vi "Set Output.vi"(8 "error in (no error)":errorcluster, 9 "Set Output":dbl, 10 "AIO_CFG":refnum<class "AIO-Configuration.lvclass">, 11 "UI Template in":refnum<class "AIO_Panel.lvclass">) -> (0 "error out":errorcluster, 3 "UI Template out":refnum<class "AIO_Panel.lvclass">)   [LabVIEW 2021, in "Simulator-Channel.lvlib" / "AIO_Panel.lvlib" / "AIO_Panel.lvclass"]
uses:
  AIO_Panel.lvclass
  Dependencies/AIO-Channel.lvlibp/Channels/AIO-Channel/AIO-Configuration_class/AIO-Configuration.lvclass
  C:/Users/averna/Documents/LV Gym DEMO/Factory Pattern/Device Channels/Dependencies/AIO-Channel.lvlibp/Generic Channel/Channel/Configuration_class/Configuration.lvclass
  tdef/info.ctl
  AIO_Panel.lvclass/AIO_Panel.ctl
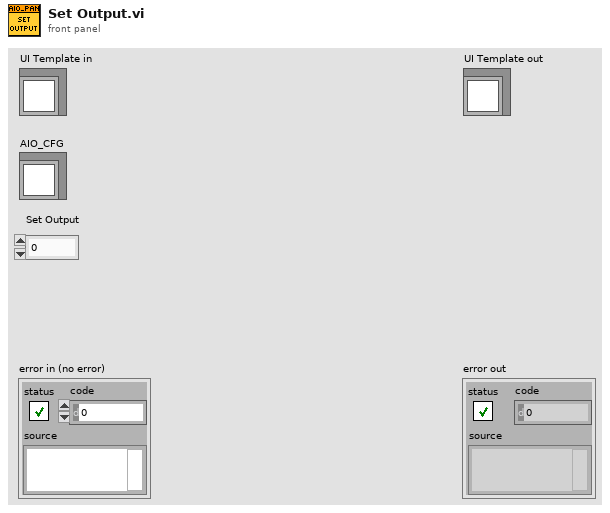
[diagram p1: front panel]
types:
  T1 = typedef "Simulator-Channel.lvlib/AIO_Panel.lvlib/AIO_Panel.lvclass/info.ctl" = cluster{"Name":string, "Numeric":dbl, "Unit":string}
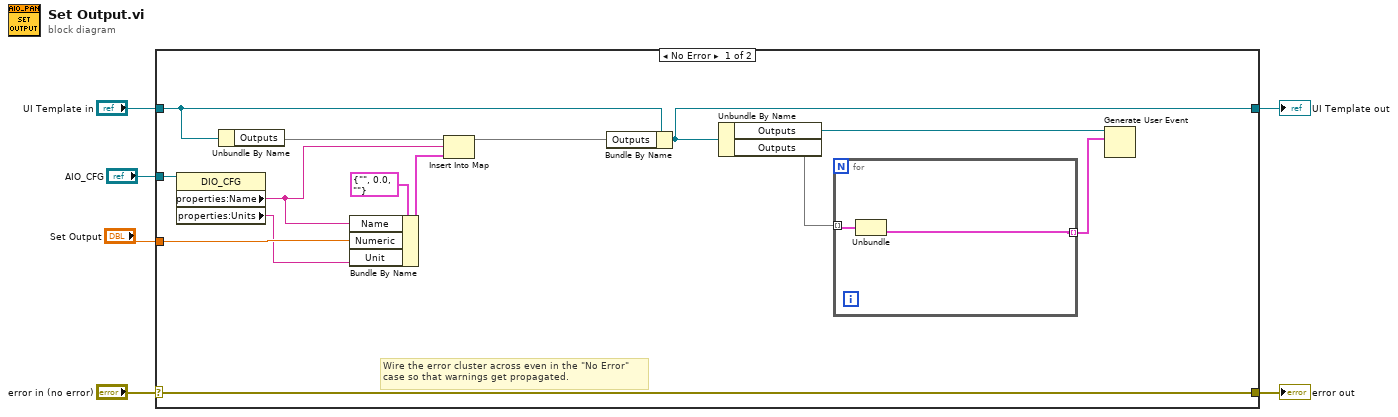
[diagram p0: block diagram]
diagram:
  n1 = case shown="No Error" "error in (no error)" {
    selector: "error in (no error)" -> [w20 w24]
    tunnel: [w20 w24] -> w5
    tunnel: [w15 w23] -> w3
    tunnel: "UI Template in" -> [w19 w23]
    tunnel: "Set Output" -> [w8 _]
    tunnel: "AIO_CFG" -> [w16 _]
    frame No Error {
      # "Wire the error cluster across even in the \"No Error\"\ncase so that warnings get propagated."
      n2 = property class="DIO_CFG"(reference=w16) -> ("properties:Name"=w9:string, "properties:Units"=w7:string)  [unwired: 1 in, 2 out]
      n3 = Unbundle By Name(w19) -> ("Outputs"=w18:map{string, T1})
      n4 = Bundle By Name(cluster=T1 {"Name"="", "Numeric"=0.0, "Unit"=""} ("value"), "Name"=w9, "Numeric"=w8, "Unit"=w7) -> (w10:T1)
      n5 = Insert Into Map(map in=w18, key=w9, value=w10) -> (map out=w17:map{string, T1})  [unwired: 2 out]
      n6 = Bundle By Name(cluster=w19, "Outputs"=w17) -> (w15:refnum<class "AIO_Panel.lvclass">)
      n7 = Unbundle By Name(w15) -> ("Outputs"=w13:refnum<user-event>, "Outputs"=w14:map{string, T1})
      n8 = for {
        tunnel: w14 -> [w22] mode=indexing
        tunnel: [w21] -> w12 mode=indexing
        n9 = Unbundle(w22) -> ("Info"=w21:T1)  [unwired: 1 out]
      }
      n10 = Generate User Event(user event=w13, event data cluster=w12) -> ()  [unwired: 2 in, 2 out]
    }
    frame Error {
    }
  }
  "error out" <- w5
  "UI Template out" <- w3
